vi "parse file string.vi"(8 "error in":errorcluster, 11 "data string":string) -> (0 "error out":errorcluster, 3 "file format":T1)   [LabVIEW 2013, in "PLConfigurationSerializer.lvlib"]
uses:
  PLConfigurationSerializer.lvlib
  file format.ctl
  <vilib>/NI/Configuration Framework/serializable configuration/NISE_CEF_serializable configuration.lvclass
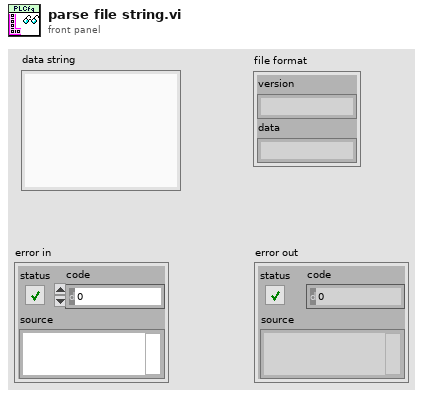
[diagram p1: front panel]
types:
  T1 = typedef "PLConfigurationSerializer.lvlib/file format.ctl" = cluster{"version":string, "data":string}
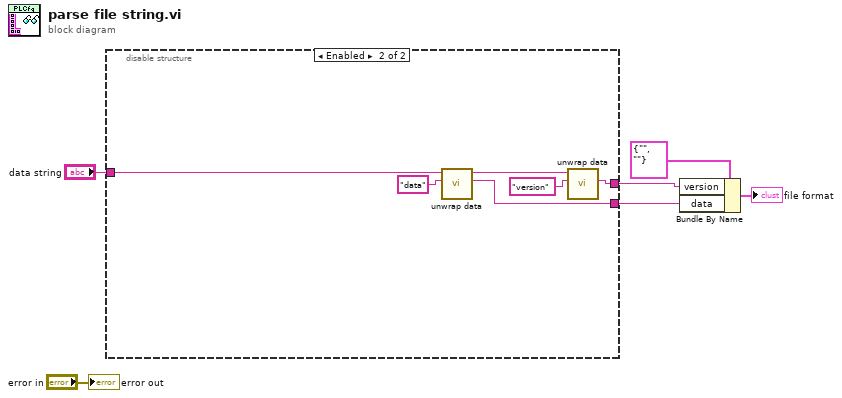
[diagram p0: block diagram]
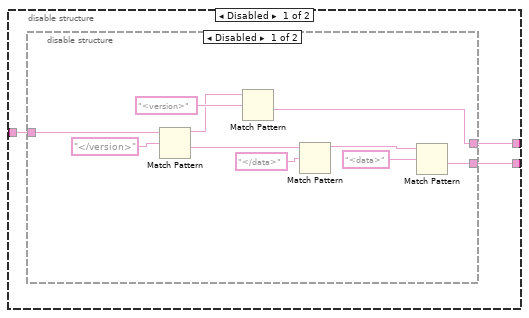
[diagram p2: hidden frame]
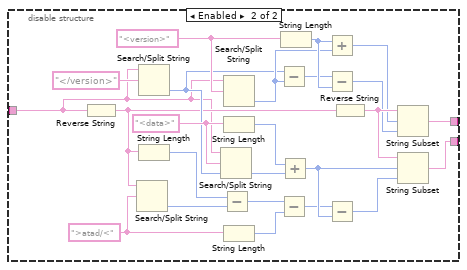
[diagram p3: hidden frame]
diagram:
  n1 = disable-structure shown="Enabled" {
    disable-tunnel: [w9 w45] -> w3
    disable-tunnel: [w8 w44] -> w2
    disable-tunnel: "data string" -> [w7 w49]
    frame Disabled {
      n2 = disable-structure shown="Disabled" {
        disable-tunnel: [w14 w20] -> w9
        disable-tunnel: [w13 w21] -> w8
        disable-tunnel: w7 -> [w10 w22]
        frame Disabled {
          n3 = Match Pattern(string=w10, regular expression="</version>") -> (before substring=w15:string, after substring=w11:string)  [unwired: 1 in, 2 out]
          n4 = Match Pattern(string=w15, regular expression="<version>") -> (after substring=w14:string)  [unwired: 1 in, 3 out]
          n5 = Match Pattern(string=w11, regular expression="</data>") -> (before substring=w12:string)  [unwired: 1 in, 3 out]
          n6 = Match Pattern(string=w12, regular expression="<data>") -> (after substring=w13:string)  [unwired: 1 in, 3 out]
        }
        frame Enabled {
          w41 = ">atad/<" ("regular expression")
          w34 = "<data>" ("regular expression")
          w31 = "<version>" ("regular expression")
          n7 = Reverse String(1:w22) -> (0:w25:string)
          n8 = Search/Split String(string=w25, search string/char (-)=w41) -> (offset of match=w36:i32)  [unwired: 1 in, 2 out]
          n9 = Search/Split String(string=w22, search string/char (-)="</version>" ("regular expression")) -> (offset of match=w29:i32)  [unwired: 1 in, 2 out]
          n10 = String Length(string=w25) -> (length=w35:i32)
          n11 = Search/Split String(string=w22, search string/char (-)=w34, offset (0)=w29) -> (offset of match=w38:i32)  [unwired: 2 out]
          n12 = Subtract(x=w35, y=w36) -> (x-y=w37:i32)
          n13 = Search/Split String(string=w22, search string/char (-)=w31) -> (offset of match=w30:i32)  [unwired: 1 in, 2 out]
          n14 = String Length(string=w34) -> (length=w39:i32)
          n15 = String Length(string=w41) -> (length=w42:i32)
          n16 = Subtract(x=w29, y=w30) -> (x-y=w32:i32)
          n17 = Subtract(x=w37, y=w42) -> (x-y=w40:i32)
          n18 = Add(x=w39, y=w38) -> (x+y=w43:i32)
          n19 = String Length(string=w31) -> (length=w33:i32)
          n20 = Add(x=w33, y=w30) -> (x+y=w24:i32)
          n21 = Subtract(x=w32, y=w33) -> (x-y=w23:i32)
          n22 = Subtract(x=w40, y=w43) -> (x-y=w27:i32)
          n23 = Reverse String(1:w25) -> (0:w26:string)
          n24 = String Subset(string=w26, offset (0)=w24, length (rest)=w23) -> (substring=w20:string)
          n25 = String Subset(string=w26, offset (0)=w43, length (rest)=w27) -> (substring=w21:string)
        }
      }
    }
    frame Enabled {
      n26 = call <vilib>:"unwrap data.vi"("identifier"="data", "data to unwrap"=w49) -> ("unwrapped data"=w44:string, "remaining string"=w47:string)  [unwired: 8 in]
      n27 = call <vilib>:"unwrap data.vi"("identifier"="version", "data to unwrap"=w47) -> ("unwrapped data"=w45:string)  [unwired: 8 in, 1 out]
    }
  }
  n28 = Bundle By Name(cluster=T1 {"version"="", "data"=""} ("file format"), "version"=w3, "data"=w2) -> (→"file format":T1)
  "error out" <- "error in"
